vi "LTE check Band Status.vi"(8 "error in (no error)":errorcluster caption="에러 입력(에러 없음)", 9 "BandWidth":T1, 10 "UL Channel":i32, 11 "Instrument Manager 입력":refnum<class "Instrument Manager.lvclass">) -> (0 "error out":errorcluster caption="에러 출력", 2 "불리언":bool, 3 "Instrument Manager 출력":refnum<class "Instrument Manager.lvclass">)   [LabVIEW 2023, in "Instrument Manager.lvclass"]
uses:
  Instrument Manager.lvclass
  Instrument Manager.lvclass/Instrument Manager.ctl
  Module/ANRITSU Call Box/Type Definition/LTE Supported BandWidth.ctl
  Module/ANRITSU Call Box/ANRITSU Call Box.lvlib
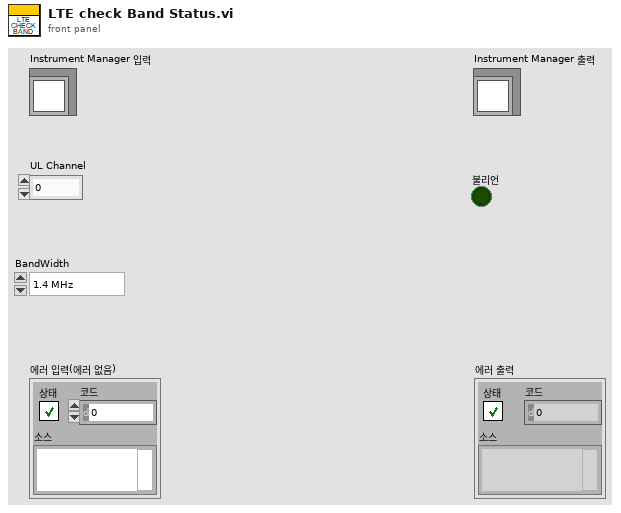
[diagram p1: front panel]
types:
  T1 = typedef "ANRITSU Call Box.lvlib/LTE Supported BandWidth.ctl" = enum16{"1.4 MHz", "3 MHz", "5 MHz", "10 MHz", "15 MHz", "20 MHz"}
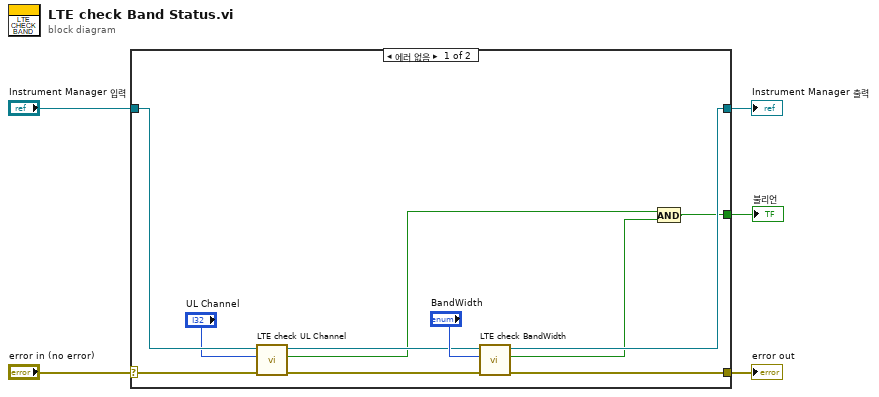
[diagram p0: block diagram]
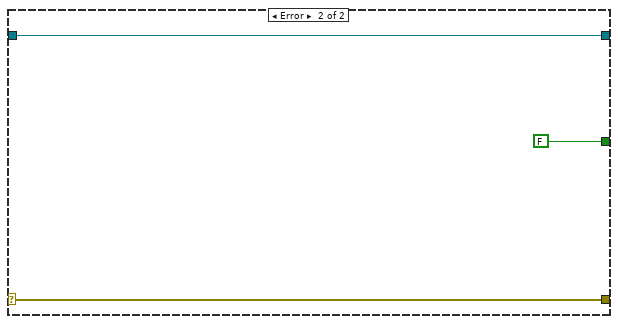
[diagram p2: hidden frame]
diagram:
  n1 = case shown="에러 없음" "error in (no error)" {
    selector: "error in (no error)" -> [w16 w19]
    tunnel: [w14 w19] -> w4
    tunnel: [w8 w18] -> w2
    tunnel: "Instrument Manager 입력" -> [w13 w18]
    tunnel: [w6 FALSE] -> w1
    frame No Error {
      n2 = call "LTE check UL Channel.vi"("error in (no error)"=w16, "UL Channel"="UL Channel", "Instrument Manager 입력"=w13) -> ("error out"=w15:errorcluster, "불리언"=w9:bool, "Instrument Manager 출력"=w10:refnum<class "Instrument Manager.lvclass">)  [unwired: 6 in]
      n3 = call "LTE check BandWidth.vi"("error in (no error)"=w15, "BandWidth"="BandWidth", "Instrument Manager 입력"=w10) -> ("error out"=w14:errorcluster, "불리언"=w7:bool, "Instrument Manager 출력"=w8:refnum<class "Instrument Manager.lvclass">)  [unwired: 6 in]
      n4 = And(x=w9, y=w7) -> (x .and. y?=w6:bool)
    }
    frame Error {
    }
  }
  "error out" <- w4
  "Instrument Manager 출력" <- w2
  "불리언" <- w1
